vi "MRC Ds Comms Get Control Data With Joysticks.vi"(8 "error in (no error)":errorcluster) -> (0 "error out":errorcluster, 2 "joystickData out":T1, 3 "data out":T2)   [LabVIEW 2023, in "MrcLib.lvlib"]
doc: "MRC_Status MRC_CALLCONV MRC_DsComms_GetControlDataWithJoysticks(struct MRC_ControlData* data, struct MRC_Joysticks* joystickData);"
uses:
  <vilib>/MRC/MrcLib.lvlib
  <vilib>/MRC/MrcLib/VIs/DS Comms/MRC_ControlData.ctl
  <vilib>/MRC/Types/MRC Str64.ctl
  <vilib>/MRC/MrcLib/VIs/DS Comms/MRC_Joysticks.ctl
  MrcLib.so
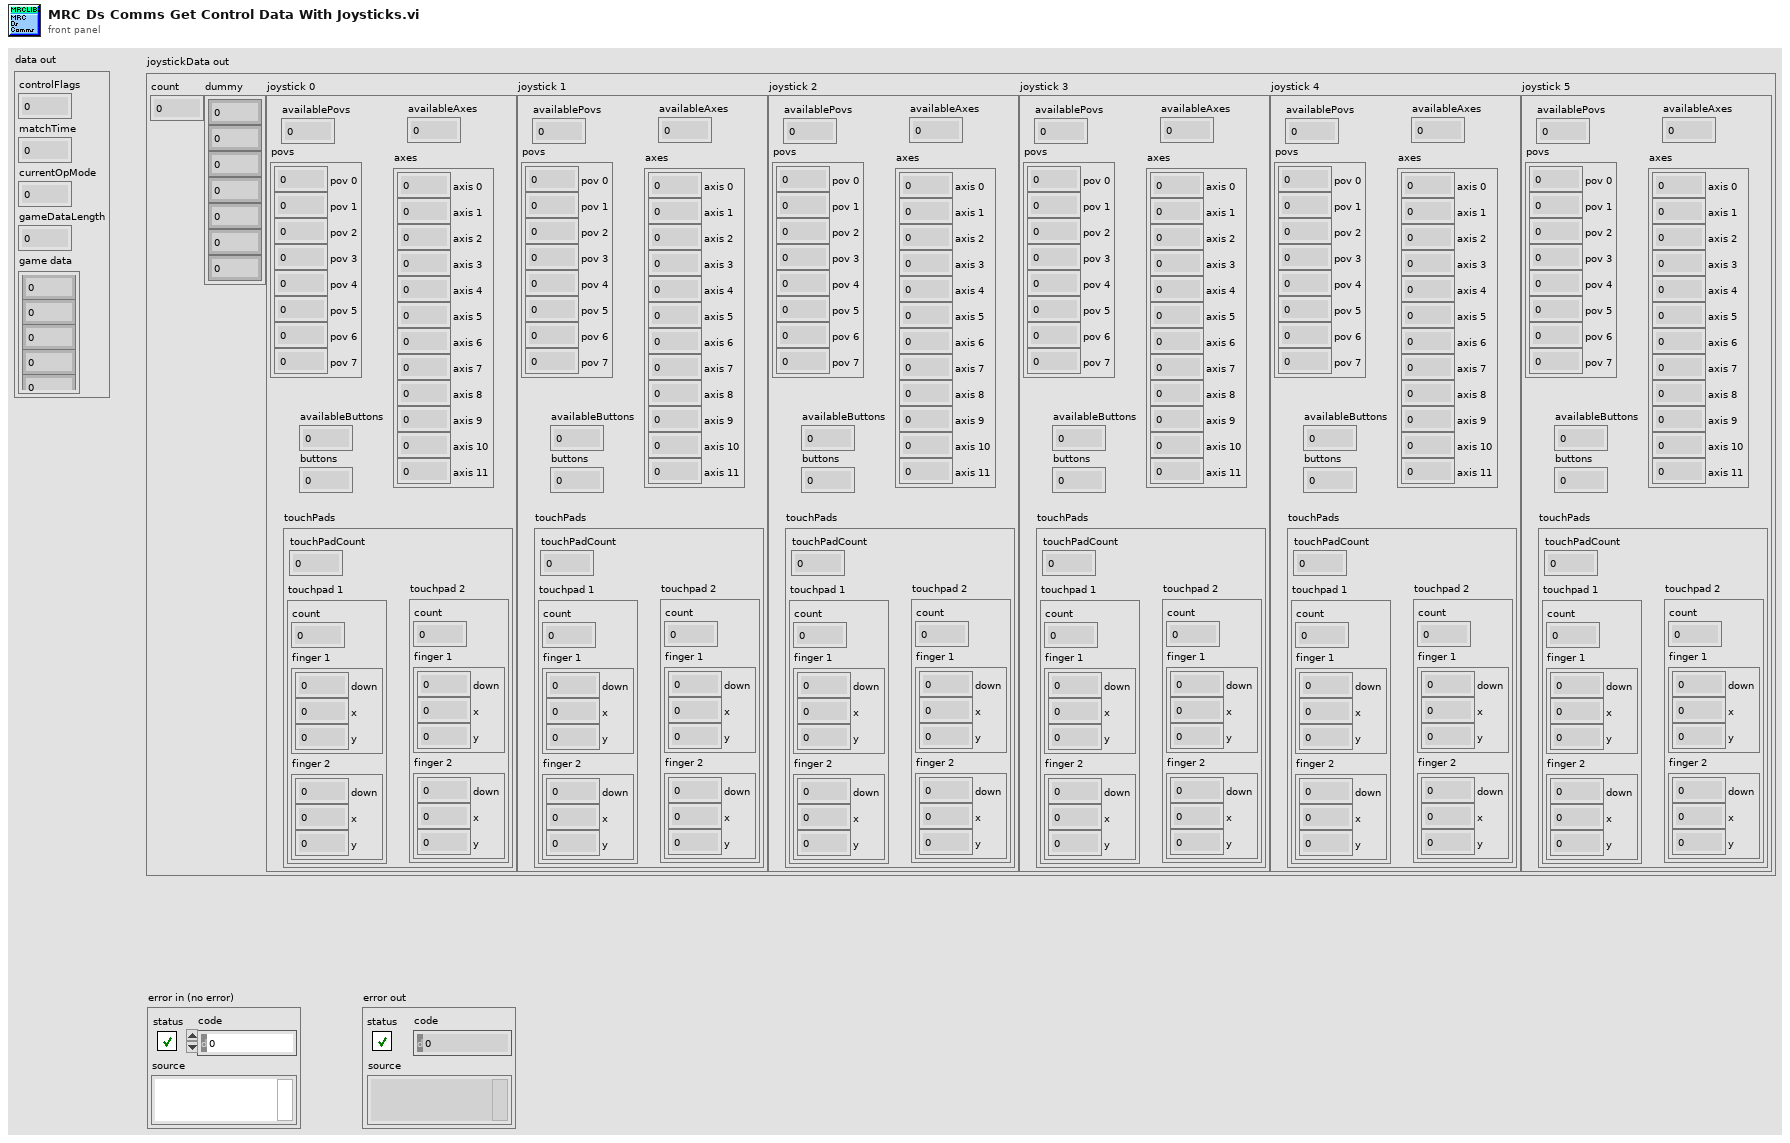
[diagram p1: front panel]
types:
  T1 = typedef "MrcLib.lvlib/MRC_Joysticks.ctl" = cluster{"count":u8, "dummy":cluster{i8, i8, i8, i8, i8, i8, i8}, "joystick 0":cluster{"availablePovs":u8, "povs":cluster{"pov 0":u8, "pov 1":u8, "pov 2":u8, "pov 3":u8, "pov 4":u8, "pov 5":u8, "pov 6":u8, "pov 7":u8}, "availableAxes":u16, "axes":cluster{"axis 0":i16, "axis 1":i16, "axis 2":i16, "axis 3":i16, "axis 4":i16, "axis 5":i16, "axis 6":i16, "axis 7":i16, "axis 8":i16, "axis 9":i16, "axis 10":i16, "axis 11":i16}, "availableButtons":u64, "buttons":u64, "touchPads":cluster{"touchPadCount":u8, "touchpad 1":cluster{"count":u8, "finger 1":cluster{"down":u8, "x":u16, "y":u16}, "finger 2":cluster{"down":u8, "x":u16, "y":u16}}, "touchpad 2":cluster{"count":u8, "finger 1":cluster{"down":u8, "x":u16, "y":u16}, "finger 2":cluster{"down":u8, "x":u16, "y":u16}}}}, "joystick 1":cluster{"availablePovs":u8, "povs":cluster{"pov 0":u8, "pov 1":u8, "pov 2":u8, "pov 3":u8, "pov 4":u8, "pov 5":u8, "pov 6":u8, "pov 7":u8}, "availableAxes":u16, "axes":cluster{"axis 0":i16, "axis 1":i16, "axis 2":i16, "axis 3":i16, "axis 4":i16, "axis 5":i16, "axis 6":i16, "axis 7":i16, "axis 8":i16, "axis 9":i16, "axis 10":i16, "axis 11":i16}, "availableButtons":u64, "buttons":u64, "touchPads":cluster{"touchPadCount":u8, "touchpad 1":cluster{"count":u8, "finger 1":cluster{"down":u8, "x":u16, "y":u16}, "finger 2":cluster{"down":u8, "x":u16, "y":u16}}, "touchpad 2":cluster{"count":u8, "finger 1":cluster{"down":u8, "x":u16, "y":u16}, "finger 2":cluster{"down":u8, "x":u16, "y":u16}}}}, "joystick 2":cluster{"availablePovs":u8, "povs":cluster{"pov 0":u8, "pov 1":u8, "pov 2":u8, "pov 3":u8, "pov 4":u8, "pov 5":u8, "pov 6":u8, "pov 7":u8}, "availableAxes":u16, "axes":cluster{"axis 0":i16, "axis 1":i16, "axis 2":i16, "axis 3":i16, "axis 4":i16, "axis 5":i16, "axis 6":i16, "axis 7":i16, "axis 8":i16, "axis 9":i16, "axis 10":i16, "axis 11":i16}, "availableButtons":u64, "buttons":u64, "touchPads":cluster{"touchPadCount":u8, "touchpad 1":cluster{"count":u8, "finger 1":cluster{"down":u8, "x":u16, "y":u16}, "finger 2":cluster{"down":u8, "x":u16, "y":u16}}, "touchpad 2":cluster{"count":u8, "finger 1":cluster{"down":u8, "x":u16, "y":u16}, "finger 2":cluster{"down":u8, "x":u16, "y":u16}}}}, "joystick 3":cluster{"availablePovs":u8, "povs":cluster{"pov 0":u8, "pov 1":u8, "pov 2":u8, "pov 3":u8, "pov 4":u8, "pov 5":u8, "pov 6":u8, "pov 7":u8}, "availableAxes":u16, "axes":cluster{"axis 0":i16, "axis 1":i16, "axis 2":i16, "axis 3":i16, "axis 4":i16, "axis 5":i16, "axis 6":i16, "axis 7":i16, "axis 8":i16, "axis 9":i16, "axis 10":i16, "axis 11":i16}, "availableButtons":u64, "buttons":u64, "touchPads":cluster{"touchPadCount":u8, "touchpad 1":cluster{"count":u8, "finger 1":cluster{"down":u8, "x":u16, "y":u16}, "finger 2":cluster{"down":u8, "x":u16, "y":u16}}, "touchpad 2":cluster{"count":u8, "finger 1":cluster{"down":u8, "x":u16, "y":u16}, "finger 2":cluster{"down":u8, "x":u16, "y":u16}}}}, "joystick 4":cluster{"availablePovs":u8, "povs":cluster{"pov 0":u8, "pov 1":u8, "pov 2":u8, "pov 3":u8, "pov 4":u8, "pov 5":u8, "pov 6":u8, "pov 7":u8}, "availableAxes":u16, "axes":cluster{"axis 0":i16, "axis 1":i16, "axis 2":i16, "axis 3":i16, "axis 4":i16, "axis 5":i16, "axis 6":i16, "axis 7":i16, "axis 8":i16, "axis 9":i16, "axis 10":i16, "axis 11":i16}, "availableButtons":u64, "buttons":u64, "touchPads":cluster{"touchPadCount":u8, "touchpad 1":cluster{"count":u8, "finger 1":cluster{"down":u8, "x":u16, "y":u16}, "finger 2":cluster{"down":u8, "x":u16, "y":u16}}, "touchpad 2":cluster{"count":u8, "finger 1":cluster{"down":u8, "x":u16, "y":u16}, "finger 2":cluster{"down":u8, "x":u16, "y":u16}}}}, "joystick 5":cluster{"availablePovs":u8, "povs":cluster{"pov 0":u8, "pov 1":u8, "pov 2":u8, "pov 3":u8, "pov 4":u8, "pov 5":u8, "pov 6":u8, "pov 7":u8}, "availableAxes":u16, "axes":cluster{"axis 0":i16, "axis 1":i16, "axis 2":i16, "axis 3":i16, "axis 4":i16, "axis 5":i16, "axis 6":i16, "axis 7":i16, "axis 8":i16, "axis 9":i16, "axis 10":i16, "axis 11":i16}, "availableButtons":u64, "buttons":u64, "touchPads":cluster{"touchPadCount":u8, "touchpad 1":cluster{"count":u8, "finger 1":cluster{"down":u8, "x":u16, "y":u16}, "finger 2":cluster{"down":u8, "x":u16, "y":u16}}, "touchpad 2":cluster{"count":u8, "finger 1":cluster{"down":u8, "x":u16, "y":u16}, "finger 2":cluster{"down":u8, "x":u16, "y":u16}}}}}
  T2 = typedef "MrcLib.lvlib/MRC_ControlData.ctl" = cluster{"controlFlags":u32, "matchTime":u16, "currentOpMode":u64, "gameDataLength":u8, "game data":T3}
  T3 = typedef "MRC Str64.ctl" = cluster{"[0]":u8, "[1]":u8, "[2]":u8, "[3]":u8, "[4]":u8, "[5]":u8, "[6]":u8, "[7]":u8, "[8]":u8, "[9]":u8, "[10]":u8, "[11]":u8, "[12]":u8, "[13]":u8, "[14]":u8, "[15]":u8, "[16]":u8, "[17]":u8, "[18]":u8, "[19]":u8, "[20]":u8, "[21]":u8, "[22]":u8, "[23]":u8, "[24]":u8, "[25]":u8, "[26]":u8, "[27]":u8, "[28]":u8, "[29]":u8, "[30]":u8, "[31]":u8, "[32]":u8, "[33]":u8, "[34]":u8, "[35]":u8, "[36]":u8, "[37]":u8, "[38]":u8, "[39]":u8, "[40]":u8, "[41]":u8, "[42]":u8, "[43]":u8, "[44]":u8, "[45]":u8, "[46]":u8, "[47]":u8, "[48]":u8, "[49]":u8, "[50]":u8, "[51]":u8, "[52]":u8, "[53]":u8, "[54]":u8, "[55]":u8, "[56]":u8, "[57]":u8, "[58]":u8, "[59]":u8, "[60]":u8, "[61]":u8, "[62]":u8, "[63]":u8}
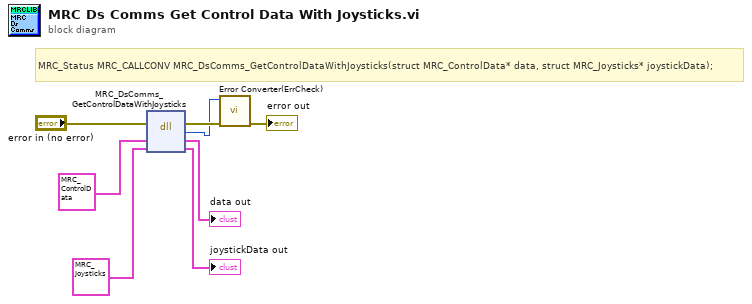
[diagram p0: block diagram]
diagram:
  # "MRC_Status MRC_CALLCONV MRC_DsComms_GetControlDataWithJoysticks(struct MRC_ControlData* data, struct MRC_Joysticks* joystickData);"
  n1 = dll-call lib="MrcLib.*" fn="MRC_DsComms_GetControlDataWithJoysticks"(error in="error in (no error)", "data"=T2 {"controlFlags"=0, "matchTime"=0, "currentOpMode"=0, "gameDataLength"=0, "game data"={"[0]"=0, "[1]"=0, "[2]"=0, "[3]"=0, "[4]"=0, "[5]"=0, "[6]"=0, "[7]"=0, "[8]"=0, "[9]"=0, "[10]"=0, "[11]"=0, "[12]"=0, "[13]"=0, "[14]"=0, "[15]"=0, "[16]"=0, "[17]"=0, "[18]"=0, "[19]"=0, "[20]"=0, "[21]"=0, "[22]"=0, "[23]"=0, "[24]"=0, "[25]"=0, "[26]"=0, "[27]"=0, "[28]"=0, "[29]"=0, "[30]"=0, "[31]"=0, "[32]"=0, "[33]"=0, "[34]"=0, "[35]"=0, "[36]"=0, "[37]"=0, "[38]"=0, "[39]"=0, "[40]"=0, "[41]"=0, "[42]"=0, "[43]"=0, "[44]"=0, "[45]"=0, "[46]"=0, "[47]"=0, "[48]"=0, "[49]"=0, "[50]"=0, "[51]"=0, "[52]"=0, "[53]"=0, "[54]"=0, "[55]"=0, "[56]"=0, "[57]"=0, "[58]"=0, "[59]"=0, "[60]"=0, "[61]"=0, "[62]"=0, "[63]"=0}} ("data out"), "joystickData"=T1 {"count"=0, "dummy"={0, 0, 0, 0, 0, 0, 0}, "joystick 0"={"availablePovs"=0, "povs"={"pov 0"=0, "pov 1"=0, "pov 2"=0, "pov 3"=0, "pov 4"=0, "pov 5"=0, "pov 6"=0, "pov 7"=0}, "availableAxes"=0, "axes"={"axis 0"=0, "axis 1"=0, "axis 2"=0, "axis 3"=0, "axis 4"=0, "axis 5"=0, "axis 6"=0, "axis 7"=0, "axis 8"=0, "axis 9"=0, "axis 10"=0, "axis 11"=0}, "availableButtons"=0, "buttons"=0, "touchPads"={"touchPadCount"=0, "touchpad 1"={"count"=0, "finger 1"={"down"=0, "x"=0, "y"=0}, "finger 2"={"down"=0, "x"=0, "y"=0}}, "touchpad 2"={"count"=0, "finger 1"={"down"=0, "x"=0, "y"=0}, "finger 2"={"down"=0, "x"=0, "y"=0}}}}, "joystick 1"={"availablePovs"=0, "povs"={"pov 0"=0, "pov 1"=0, "pov 2"=0, "pov 3"=0, "pov 4"=0, "pov 5"=0, "pov 6"=0, "pov 7"=0}, "availableAxes"=0, "axes"={"axis 0"=0, "axis 1"=0, "axis 2"=0, "axis 3"=0, "axis 4"=0, "axis 5"=0, "axis 6"=0, "axis 7"=0, "axis 8"=0, "axis 9"=0, "axis 10"=0, "axis 11"=0}, "availableButtons"=0, "buttons"=0, "touchPads"={"touchPadCount"=0, "touchpad 1"={"count"=0, "finger 1"={"down"=0, "x"=0, "y"=0}, "finger 2"={"down"=0, "x"=0, "y"=0}}, "touchpad 2"={"count"=0, "finger 1"={"down"=0, "x"=0, "y"=0}, "finger 2"={"down"=0, "x"=0, "y"=0}}}}, "joystick 2"={"availablePovs"=0, "povs"={"pov 0"=0, "pov 1"=0, "pov 2"=0, "pov 3"=0, "pov 4"=0, "pov 5"=0, "pov 6"=0, "pov 7"=0}, "availableAxes"=0, "axes"={"axis 0"=0, "axis 1"=0, "axis 2"=0, "axis 3"=0, "axis 4"=0, "axis 5"=0, "axis 6"=0, "axis 7"=0, "axis 8"=0, "axis 9"=0, "axis 10"=0, "axis 11"=0}, "availableButtons"=0, "buttons"=0, "touchPads"={"touchPadCount"=0, "touchpad 1"={"count"=0, "finger 1"={"down"=0, "x"=0, "y"=0}, "finger 2"={"down"=0, "x"=0, "y"=0}}, "touchpad 2"={"count"=0, "finger 1"={"down"=0, "x"=0, "y"=0}, "finger 2"={"down"=0, "x"=0, "y"=0}}}}, "joystick 3"={"availablePovs"=0, "povs"={"pov 0"=0, "pov 1"=0, "pov 2"=0, "pov 3"=0, "pov 4"=0, "pov 5"=0, "pov 6"=0, "pov 7"=0}, "availableAxes"=0, "axes"={"axis 0"=0, "axis 1"=0, "axis 2"=0, "axis 3"=0, "axis 4"=0, "axis 5"=0, "axis 6"=0, "axis 7"=0, "axis 8"=0, "axis 9"=0, "axis 10"=0, "axis 11"=0}, "availableButtons"=0, "buttons"=0, "touchPads"={"touchPadCount"=0, "touchpad 1"={"count"=0, "finger 1"={"down"=0, "x"=0, "y"=0}, "finger 2"={"down"=0, "x"=0, "y"=0}}, "touchpad 2"={"count"=0, "finger 1"={"down"=0, "x"=0, "y"=0}, "finger 2"={"down"=0, "x"=0, "y"=0}}}}, "joystick 4"={"availablePovs"=0, "povs"={"pov 0"=0, "pov 1"=0, "pov 2"=0, "pov 3"=0, "pov 4"=0, "pov 5"=0, "pov 6"=0, "pov 7"=0}, "availableAxes"=0, "axes"={"axis 0"=0, "axis 1"=0, "axis 2"=0, "axis 3"=0, "axis 4"=0, "axis 5"=0, "axis 6"=0, "axis 7"=0, "axis 8"=0, "axis 9"=0, "axis 10"=0, "axis 11"=0}, "availableButtons"=0, "buttons"=0, "touchPads"={"touchPadCount"=0, "touchpad 1"={"count"=0, "finger 1"={"down"=0, "x"=0, "y"=0}, "finger 2"={"down"=0, "x"=0, "y"=0}}, "touchpad 2"={"count"=0, "finger 1"={"down"=0, "x"=0, "y"=0}, "finger 2"={"down"=0, "x"=0, "y"=0}}}}, "joystick 5"={"availablePovs"=0, "povs"={"pov 0"=0, "pov 1"=0, "pov 2"=0, "pov 3"=0, "pov 4"=0, "pov 5"=0, "pov 6"=0, "pov 7"=0}, "availableAxes"=0, "axes"={"axis 0"=0, "axis 1"=0, "axis 2"=0, "axis 3"=0, "axis 4"=0, "axis 5"=0, "axis 6"=0, "axis 7"=0, "axis 8"=0, "axis 9"=0, "axis 10"=0, "axis 11"=0}, "availableButtons"=0, "buttons"=0, "touchPads"={"touchPadCount"=0, "touchpad 1"={"count"=0, "finger 1"={"down"=0, "x"=0, "y"=0}, "finger 2"={"down"=0, "x"=0, "y"=0}}, "touchpad 2"={"count"=0, "finger 1"={"down"=0, "x"=0, "y"=0}, "finger 2"={"down"=0, "x"=0, "y"=0}}}}} ("joystickData in")) -> (error out=w3:errorcluster, "return type"=w1:i32, "data"=→"data out":T2, "joystickData"=→"joystickData out":T1)  [unwired: 2 in, 1 out]
  n2 = call <vilib>:"Error Converter(ErrCheck).vi"("error in (no error)"=w3, "status"=w1) -> ("error out"=→"error out":errorcluster)  [unwired: 9 in]
